vi "Create User Events.vi"(8 "error in (no error)":errorcluster) -> (0 "error out":errorcluster, 3 "User Events":T1)   [LabVIEW 2026, in "User Event - Stop.lvlib"]
doc: "Create a boolean user event that will be used to stop the event loop from the message handling loop.à`´"
uses:
  User Event - Stop.lvlib
  User Events.ctl
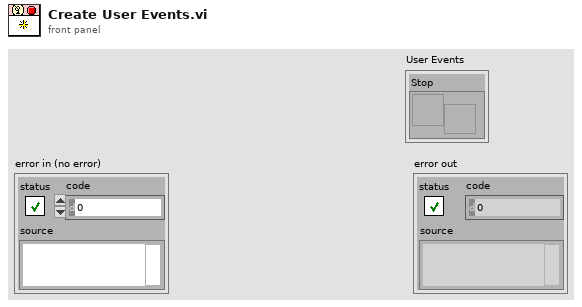
[diagram p1: front panel]
types:
  T1 = typedef "User Event - Stop.lvlib/User Events.ctl" = cluster{"Stop":refnum<user-event>}
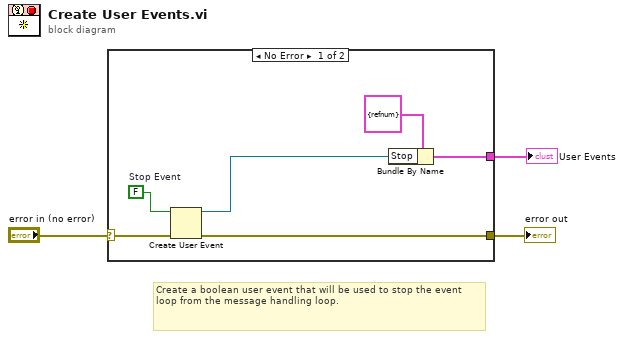
[diagram p0: block diagram]
diagram:
  # "Create a boolean user event that will be used to stop the event loop from the message handling loop."
  n1 = case shown="No Error" "error in (no error)" {
    selector: "error in (no error)" -> [w9 w10]
    tunnel: [w7 w10] -> w3
    tunnel: [w4 _] -> w1
    frame No Error {
      w8 = FALSE  # Stop Event
      n2 = Create User Event(user event datatype=w8, error in=w9) -> (user event=w5:refnum<user-event>, error out=w7:errorcluster)
      n3 = Bundle By Name(cluster=T1 {"Stop"=refnum} ("User Events"), "Stop"=w5) -> (w4:T1)
    }
    frame Error {
    }
  }
  "error out" <- w3
  "User Events" <- w1
